vi "Check IO Names.vi"(8 "prior problem":string, 9 "IO List":cluster{"name":string, "type":string}[](array[cluster]), 10 "allowed types":string[](array[string]), 11 "names":string[](array[string])) -> (3 "problem":string)   [LabVIEW 2026]
doc: "Returns prior problem unchanged if it is not empty. Otherwise names the first item that is missing from the IO list or whose type is not allowed. AF-free."
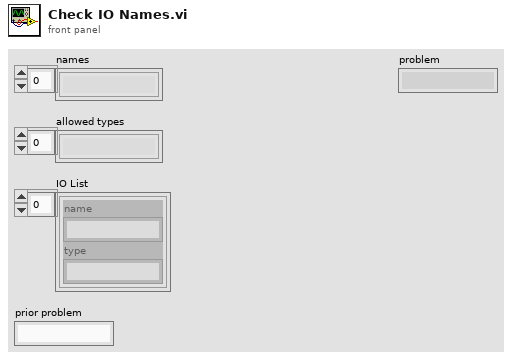
[diagram p1: front panel]
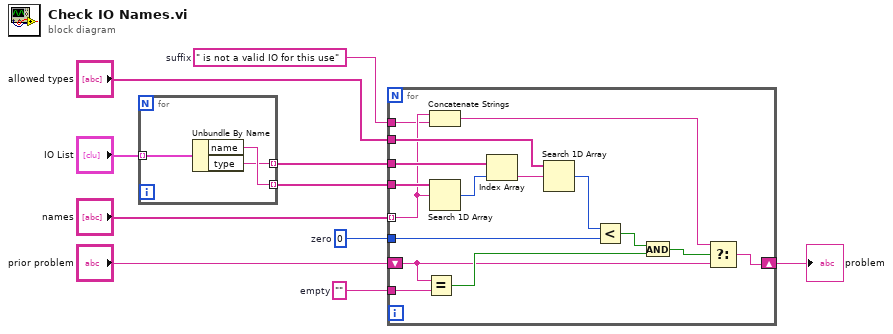
[diagram p0: block diagram]
diagram:
  w3 = " is not a valid IO for this use"  # suffix
  w4 = 0  # zero
  w5 = ""  # empty
  n1 = for {
    tunnel: "IO List" -> [w13] mode=indexing
    tunnel: [w12] -> w8 mode=indexing
    tunnel: [w11] -> w7 mode=indexing
    n2 = Unbundle By Name(w13) -> ("name"=w12:string, "type"=w11:string)
  }
  n3 = for {
    tunnel: "names" -> [w19] mode=indexing
    tunnel: w8 -> [w29]
    tunnel: w7 -> [w28]
    tunnel: "allowed types" -> [w26]
    tunnel: w5 -> [w22]
    tunnel: w4 -> [w23]
    tunnel: w3 -> [w18]
    shift-right: [w14] -> w1
    shift-left: "prior problem" -> [w15]
    n4 = Equal?(x=w15, y=w22) -> (x = y?=w20:bool)
    n5 = Concatenate Strings(w19, w18) -> (w17:string)
    n6 = Search 1D Array(1D array=w29, element=w19) -> (index of element=w27:i32)  [unwired: 1 in]
    n7 = Index Array(array=w28, index=w27) -> (element=w25:string)
    n8 = Search 1D Array(1D array=w26, element=w25) -> (index of element=w24:i32)  [unwired: 1 in]
    n9 = Less?(x=w24, y=w23) -> (x < y?=w21:bool)
    n10 = And(x=w21, y=w20) -> (x .and. y?=w16:bool)
    n11 = Select(t=w17, s=w16, f=w15) -> (s? t:f=w14:string)
  }
  "problem" <- w1
